vi "Get Page VI.vi"(8 "error in (no error)":errorcluster, 9 "GUID":string, 10 "Item Ref":T1 format="%.0x", 11 "System Explorer Dispatcher Implementation in":refnum<class "System Explorer Dispatcher.lvclass">) -> (0 "error out":errorcluster, 2 "page reference":refnum<vi>, 3 "System Explorer Dispatcher Implementation out":refnum<class "System Explorer Dispatcher.lvclass">)   [LabVIEW 2020, in "Ballard ARINC 429 System Explorer.lvlib" / "Implementation.lvlib" / "System Explorer Dispatcher.lvclass"]
uses:
  System Explorer Dispatcher.lvclass
  <vilib>/NI VeriStand/Custom Device API/Custom Device Item Ref.ctl
  Scripting/Ballard/Constants.vi
  System Explorer/Pages/Configuration Files.vi
  System Explorer/Pages/Channel Specification.vi
  System Explorer/Pages/Parameter.vi
  System Explorer/Pages/Receive Time.vi
  System Explorer/Pages/Word.vi
  System Explorer/Pages/Status Channel.vi
  System Explorer/Pages/Logging.vi
  System Explorer/Pages/Timing.vi
  Implementation.lvlib
  Scripting/Ballard/Ballard ARINC 429 Scripting.lvlib
  <vilib>/NI VeriStand/Custom Device API/Custom Device API.lvlib
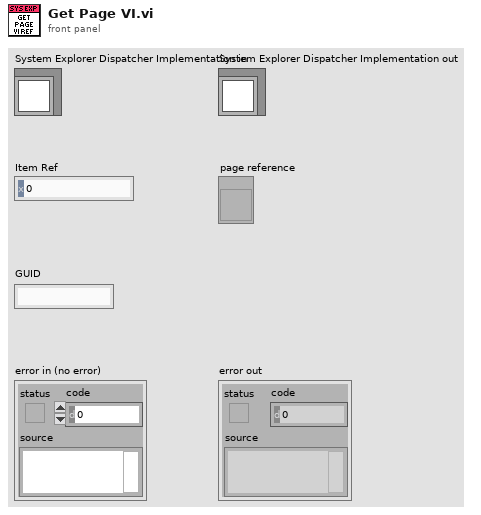
[diagram p1: front panel]
types:
  T1 = typedef "Custom Device API.lvlib/Custom Device Item Ref.ctl" = u64
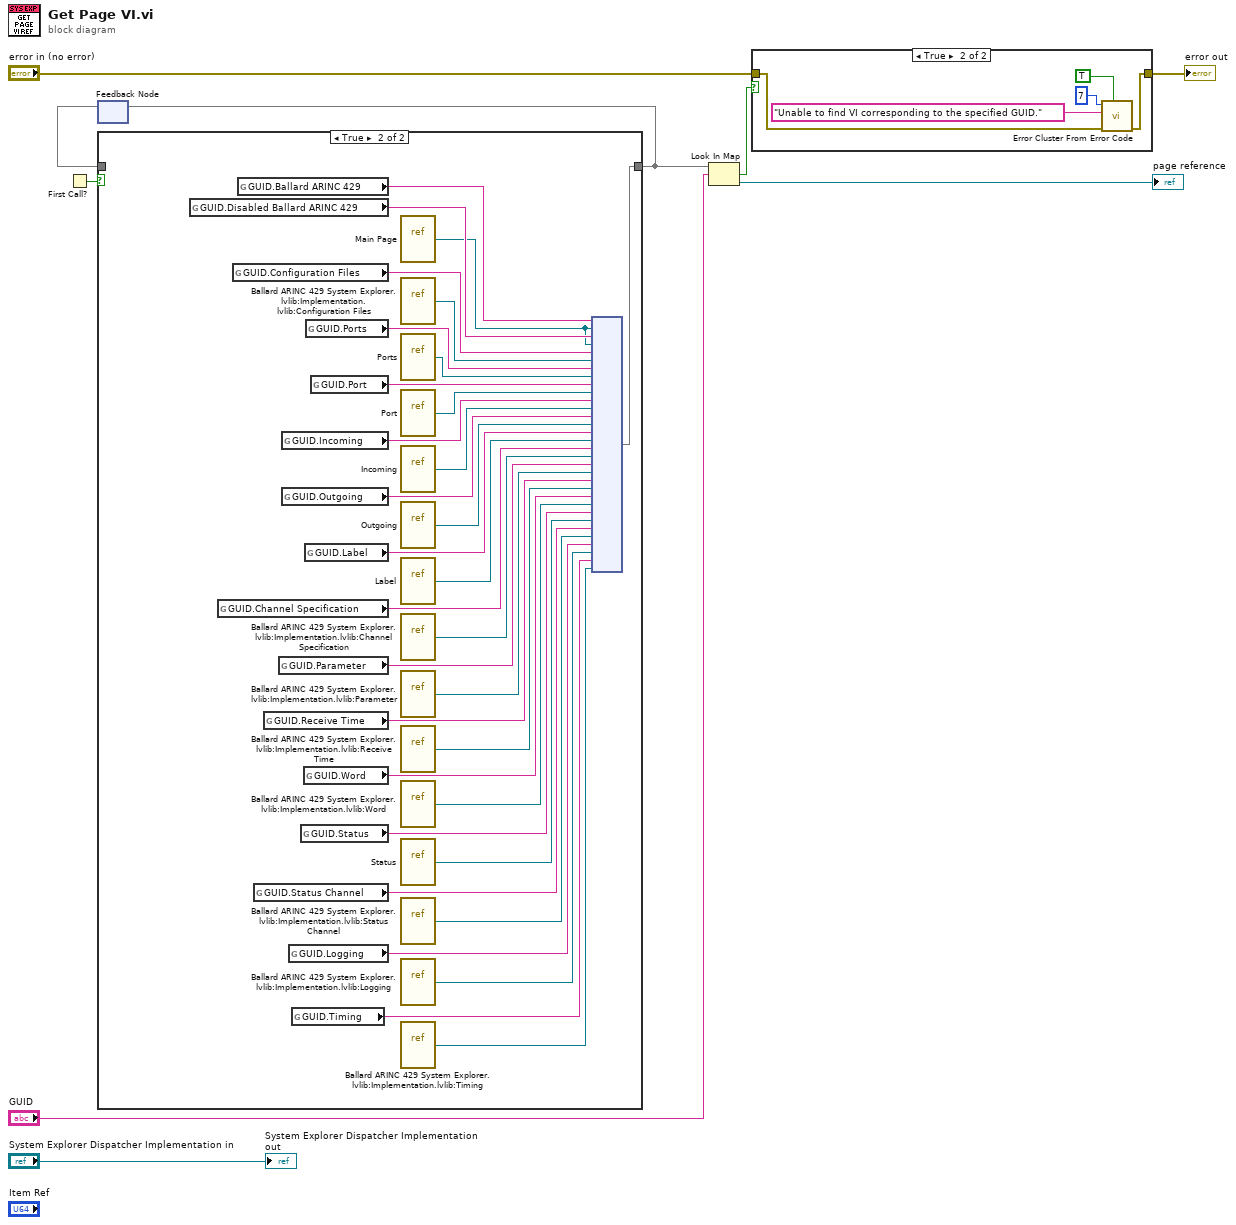
[diagram p0: block diagram]
diagram:
  n1 = First Call?() -> (First Call?: T/F=w8:bool)
  n2 = feedback #1() -> (w7:map{string, refnum<vi>})  [unwired: 1 in]
  n3 = case shown="True" w8 {
    tunnel: [w10 w42] -> w6
    tunnel: w7 -> [w10 _]
    frame False {
    }
    frame True {
      n4 = global read "Constants.vi" "GUID.Disabled Ballard ARINC 429"() -> (w14:string)
      n5 = global read "Constants.vi" "GUID.Channel Specification"() -> (w29:string)
      n6 = global read "Constants.vi" "GUID.Configuration Files"() -> (w40:string)
      n7 = global read "Constants.vi" "GUID.Ballard ARINC 429"() -> (w15:string)
      n8 = global read "Constants.vi" "GUID.Status Channel"() -> (w19:string)
      n9 = global read "Constants.vi" "GUID.Receive Time"() -> (w25:string)
      n10 = global read "Constants.vi" "GUID.Parameter"() -> (w27:string)
      n11 = global read "Constants.vi" "GUID.Incoming"() -> (w35:string)
      n12 = global read "Constants.vi" "GUID.Outgoing"() -> (w33:string)
      n13 = global read "Constants.vi" "GUID.Logging"() -> (w17:string)
      n14 = global read "Constants.vi" "GUID.Timing"() -> (w12:string)
      n15 = global read "Constants.vi" "GUID.Status"() -> (w21:string)
      n16 = global read "Constants.vi" "GUID.Word"() -> (w23:string)
      n17 = global read "Constants.vi" "GUID.Label"() -> (w31:string)
      n18 = global read "Constants.vi" "GUID.Ports"() -> (w39:string)
      n19 = global read "Constants.vi" "GUID.Port"() -> (w37:string)
      n20 = vi-ref "Main Page.vi"() -> (w13:refnum<vi>)
      n21 = vi-ref "Ballard ARINC 429 System Explorer.lvlib:Implementation.lvlib:Configuration Files.vi"() -> (w41:refnum<vi>)
      n22 = vi-ref "Ports.vi"() -> (w38:refnum<vi>)
      n23 = vi-ref "Port.vi"() -> (w36:refnum<vi>)
      n24 = vi-ref "Incoming.vi"() -> (w34:refnum<vi>)
      n25 = vi-ref "Outgoing.vi"() -> (w32:refnum<vi>)
      n26 = vi-ref "Label.vi"() -> (w30:refnum<vi>)
      n27 = vi-ref "Ballard ARINC 429 System Explorer.lvlib:Implementation.lvlib:Channel Specification.vi"() -> (w28:refnum<vi>)
      n28 = vi-ref "Ballard ARINC 429 System Explorer.lvlib:Implementation.lvlib:Parameter.vi"() -> (w26:refnum<vi>)
      n29 = vi-ref "Ballard ARINC 429 System Explorer.lvlib:Implementation.lvlib:Receive Time.vi"() -> (w24:refnum<vi>)
      n30 = vi-ref "Ballard ARINC 429 System Explorer.lvlib:Implementation.lvlib:Word.vi"() -> (w22:refnum<vi>)
      n31 = vi-ref "Status.vi"() -> (w20:refnum<vi>)
      n32 = vi-ref "Ballard ARINC 429 System Explorer.lvlib:Implementation.lvlib:Status Channel.vi"() -> (w18:refnum<vi>)
      n33 = vi-ref "Ballard ARINC 429 System Explorer.lvlib:Implementation.lvlib:Logging.vi"() -> (w16:refnum<vi>)
      n34 = vi-ref "Ballard ARINC 429 System Explorer.lvlib:Implementation.lvlib:Timing.vi"() -> (w11:refnum<vi>)
      n35 = node(w15, w13, w14, w13, w40, w41, w39, w38, w37, w36, w35, w34, w33, w32, w31, w30, w29, w28, w27, w26, w25, w24, w23, w22, w21, w20, w19, w18, w17, w16, w12, w11) -> (w42:map{string, refnum<vi>})
    }
  }
  n36 = feedback-in #1(w6) -> ()
  n37 = Look In Map(map=w6, key="GUID") -> (key not found?=w4:bool, value=→"page reference":refnum<vi>)  [unwired: 1 in]
  n38 = case shown="True" w4 {
    tunnel: [w43 w45] -> w3
    tunnel: "error in (no error)" -> [w43 w44]
    frame False {
    }
    frame True {
      n39 = call <vilib>:"Error Cluster From Error Code.vi"("show call chain? (False)"=TRUE, "error in (no error)"=w44, "error message (\"\")"="Unable to find VI corresponding to the specified GUID." ("error message (\"\")"), "error code (0)"=7) -> ("error out"=w45:errorcluster)  [unwired: 5 in]
    }
  }
  "error out" <- w3
  "System Explorer Dispatcher Implementation out" <- "System Explorer Dispatcher Implementation in"
